vi "Configure Module.vi"(8 "error in (no error)":errorcluster, 10 "IOV ref in":variant, 11 "9237 in":refnum<class "9237.lvclass">) -> (0 "error out":errorcluster, 2 "IOV ref out":variant, 3 "9237 out":refnum<class "9237.lvclass">)   [LabVIEW 2020, in "Modules.lvlib" / "9237.lvclass"]
uses:
  9237.lvclass
  <resource>/objmgr/cRIO.rc
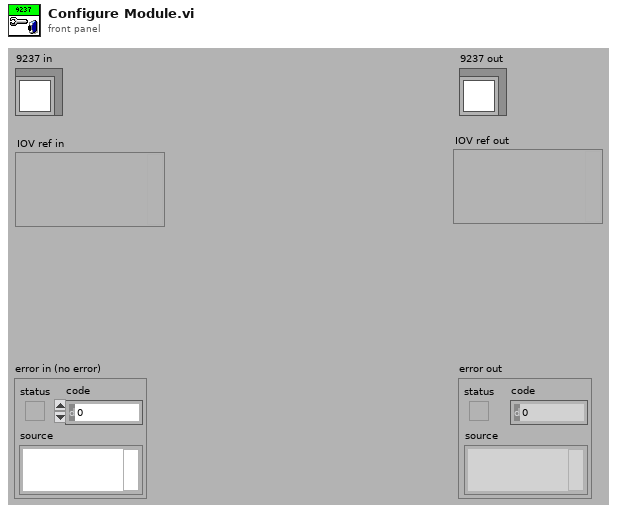
[diagram p1: front panel]
types:
  T1 = typedef "Modules.lvlib/9237.lvclass/_nicrio_cRIO-923x_ExcitationVoltageRing.ctl" = u8
  T2 = typedef "Modules.lvlib/9237.lvclass/Data rate.ctl" = u32
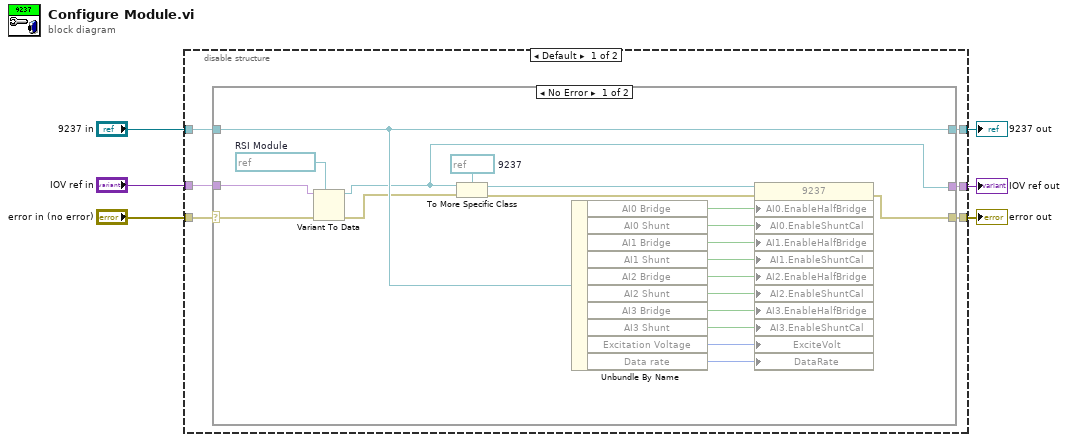
[diagram p0: block diagram]
diagram:
  n1 = disable-structure shown="Default" {
    disable-tunnel: "error in (no error)" -> [w12 w38]
    disable-tunnel: [w11 w38] -> w5
    disable-tunnel: "9237 in" -> [w10 w36]
    disable-tunnel: [w9 w36] -> w3
    disable-tunnel: "IOV ref in" -> [w8 w37]
    disable-tunnel: [w7 w37] -> w1
    frame condition #0 {
      n2 = case shown="No Error" w12 {
        selector: w12 -> [w22 w35]
        tunnel: [w20 w35] -> w11
        tunnel: [w32 w34] -> w9
        tunnel: w10 -> [w32 w34]
        tunnel: w8 -> [w15 w33]
        tunnel: [w14 w33] -> w7
        frame No Error {
          w13 = refnum<k21> refnum  # RSI Module
          w23 = refnum<k21> refnum  # 9237
          n3 = Variant To Data(error in=w22, type=w13, Variant=w15) -> (data=w14:refnum<k21>, error out=w16:errorcluster)
          n4 = To More Specific Class(target class=w23, reference=w14, error in=w16) -> (specific class reference=w18:refnum<k21>, error out=w21:errorcluster)
          n5 = Unbundle By Name(w32) -> ("AI0 Bridge"=w31:bool, "AI0 Shunt"=w30:bool, "AI1 Bridge"=w29:bool, "AI1 Shunt"=w28:bool, "AI2 Bridge"=w27:bool, "AI2 Shunt"=w26:bool, "AI3 Bridge"=w25:bool, "AI3 Shunt"=w24:bool, "Excitation Voltage"=w19:T1, "Data rate"=w17:T2)
          n6 = property class="9237"(reference=w18, error in=w21, "AI0.EnableHalfBridge"=w31, "AI0.EnableShuntCal"=w30, "AI1.EnableHalfBridge"=w29, "AI1.EnableShuntCal"=w28, "AI2.EnableHalfBridge"=w27, "AI2.EnableShuntCal"=w26, "AI3.EnableHalfBridge"=w25, "AI3.EnableShuntCal"=w24, "ExciteVolt"=w19, "DataRate"=w17) -> (error out=w20:errorcluster)  [unwired: 1 out]
        }
        frame Error {
        }
      }
    }
    frame condition #1 (active) {
    }
  }
  "error out" <- w5
  "9237 out" <- w3
  "IOV ref out" <- w1
